vi "Generate VI Name.vi"(8 "error in":errorcluster, 11 "Python Function Name":string) -> (0 "error out":errorcluster, 3 "VI Name":string)   [LabVIEW 2026]
doc: "This VI generates a display-friendly VI name from a python function name by converting underscore-separated text into proper case words."
uses:
  <userlib>/_OpenG.lib/string/string.llb/To Proper Case (String)__ogtk.vi
  <vilib>/regexp/Match Regular Expression.xnode
  <userlib>/_OpenG.lib/string/string.llb/openg_string.lvlib
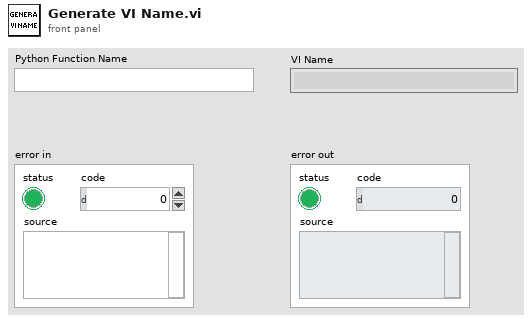
[diagram p1: front panel]
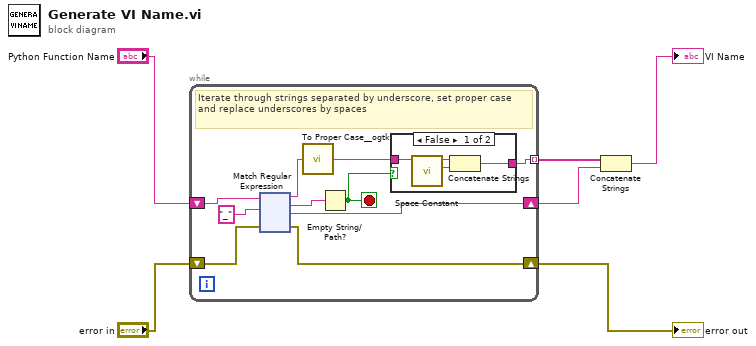
[diagram p0: block diagram]
diagram:
  n1 = while {
    shift-right: [w15] -> w5
    shift-left: "error in" -> [w16]
    shift-right: [w12] -> w3
    shift-left: "Python Function Name" -> [w14]
    tunnel: [w8] -> w4 mode=indexing
    stop <- w7 stop-if-true
    # "Iterate through strings separated by underscore, set proper case and replace underscores by spaces"
    n2 = xnode "Match Regular Expression"("input string"=w14, "regular expression"="_", "error in"=w16) -> ("before match"=w11:string, "whole match"=w10:string, "after match"=w12:string, "error out"=w15:errorcluster)  [unwired: 3 in, 1 out]
    n3 = call-poly <userlib>:"To Proper Case__ogtk.vi"("string"=w11) -> ("proper case string"=w9:string)  [unwired: 4 in]
    n4 = Empty String/Path?(string/path=w10) -> (empty?=w7:bool)
    n5 = case shown="False" w7 {
      tunnel: w9 -> [w19 w20]
      tunnel: [w18 w20] -> w8
      frame False {
        n6 = call <vilib>:"Space Constant.vi"() -> ("String"=w17:string)
        n7 = Concatenate Strings(w19, w17) -> (w18:string)
      }
      frame True {
      }
    }
  }
  "error out" <- w5
  n8 = Concatenate Strings(w4, w3) -> (→"VI Name":string)
